vi "Each Base Sequence Analysis.vi"(11 "Sample Sequence":string) -> (0 "Each Base Sequence Info":T1, 1 "Base IDX vs S# Matrix":bool[][](array[boolean]), 2 "Cutted Sequence":string, 3 "Base (n)":i32)   [LabVIEW 2018]
panel:
  out "Base Species IDX":i32[](array[numeric])
  out "Base Sequence Array":string[](array[string])
  out "5'→3' location Number":i32[](array[numeric])
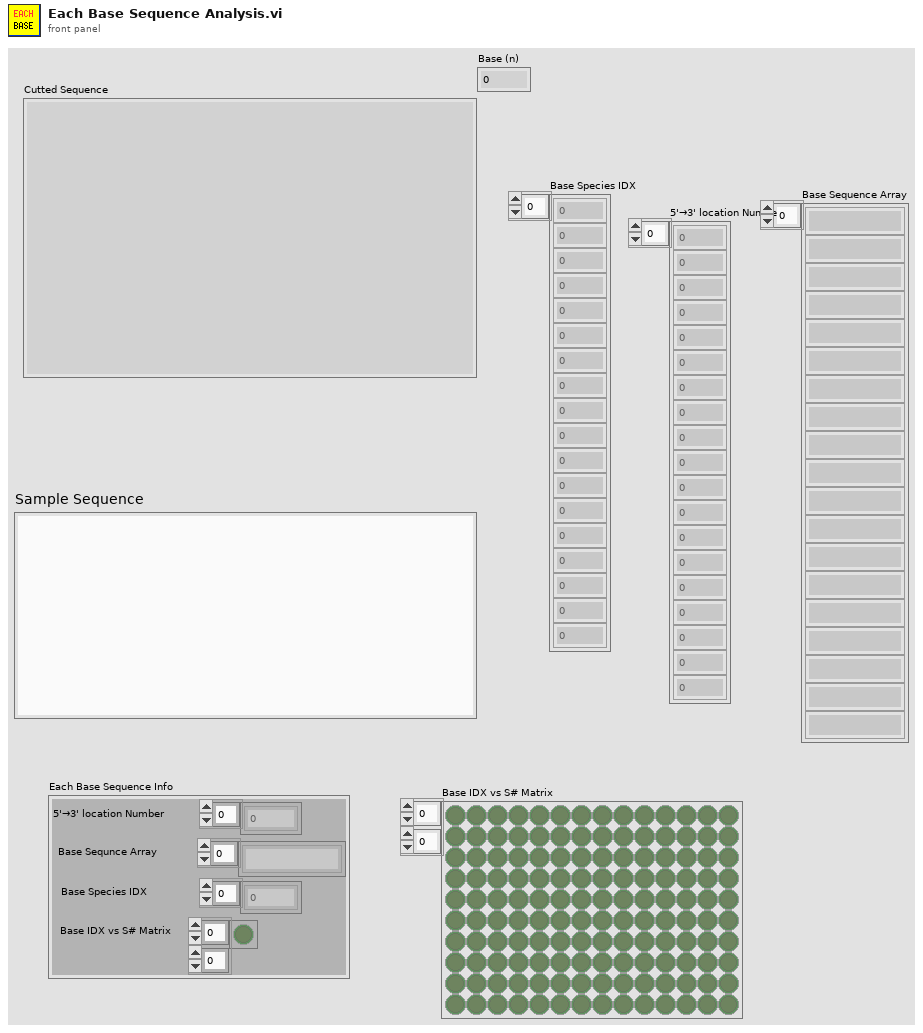
[diagram p1: front panel]
types:
  T1 = cluster{"5'→3' location Number":i32[], "Base Sequnce Array":string[], "Base Species IDX":i32[], "Base IDX vs S# Matrix":bool[][]}
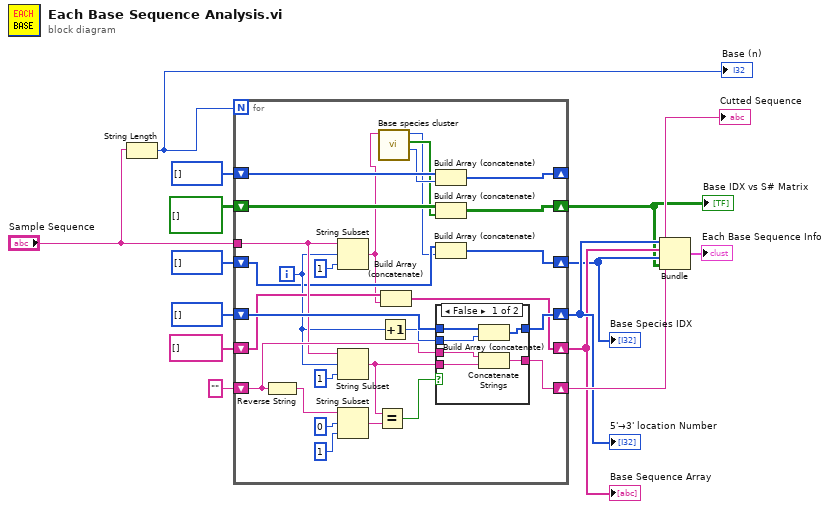
[diagram p0: block diagram]
diagram:
  n1 = String Length(string="Sample Sequence") -> (length=w14:i32)
  "Base (n)" <- w14
  n2 = for {
    N: w14 -> [_]
    tunnel: "Sample Sequence" -> [w29]
    shift-right: [w38] -> w12
    shift-left: "" -> [w37]
    shift-right: [w32] -> w7
    shift-left: i32[] [] -> [w31]
    shift-right: [w27] -> w6
    shift-left: string[] [] -> [w26]
    shift-right: [w24] -> w5
    shift-left: i32[] [] -> [w23]
    shift-right: [w22] -> w4
    shift-left: bool[][] [] -> [w21]
    shift-right: [w20] -> _
    shift-left: u32[] [] -> [w19]
    i -> [w25]
    n3 = Reverse String(1:w37) -> (0:w36:string)
    n4 = String Subset(string=w29, offset (0)=w25, length (rest)=1 ("長さ（残り）")) -> (substring=w18:string)
    n5 = String Subset(string=w29, offset (0)=w25, length (rest)=1 ("長さ（残り）")) -> (substring=w39:string)
    n6 = String Subset(string=w36, offset (0)=0 ("オフセット（0）"), length (rest)=1 ("長さ（残り）")) -> (substring=w35:string)
    n7 = Equal?(x=w39, y=w35) -> (x = y?=w40:bool)
    n8 = call "Base species cluster.vi"("Base"=w18) -> ("Base Color"=w17:u32, "Base Array"=w16:bool[], "Base Species IDX"=w15:i32)  [unwired: 6 in, 2 out]
    n9 = Increment(x=w25) -> (x+1=w30:i32)
    n10 = Build Array (concatenate)(w26, w18) -> (w27:string[])
    n11 = Build Array (concatenate)(w19, w17) -> (w20:u32[])
    n12 = Build Array (concatenate)(w21, w16) -> (w22:bool[][])
    n13 = Build Array (concatenate)(w23, w15) -> (w24:i32[])
    n14 = case shown="False" w40 {
      tunnel: w39 -> [w47 _]
      tunnel: [w46 w49] -> w38
      tunnel: w37 -> [w45 w49]
      tunnel: w30 -> [w43 _]
      tunnel: [w44 w48] -> w32
      tunnel: w31 -> [w42 w48]
      frame False {
        n15 = Build Array (concatenate)(w42, w43) -> (w44:i32[])
        n16 = Concatenate Strings(w45, w47) -> (w46:string)
      }
      frame True {
      }
    }
  }
  "Cutted Sequence" <- w12
  "5'→3' location Number" <- w7
  "Base Sequence Array" <- w6
  "Base Species IDX" <- w5
  "Base IDX vs S# Matrix" <- w4
  n17 = Bundle(w7, w6, w5, w4) -> (→"Each Base Sequence Info":cluster{i32[], string[], i32[], bool[][]})  [unwired: 1 in]
